vi "Convert Device Status.vi"(11 "device status":T4) -> (3 "CAN Status":T1)   [LabVIEW 2021, in "CAN RW CANsub.lvclass"]
doc: "It converts the device status to the CIF type CAN Status."
uses:
  CAN RW CANsub.lvclass
  <vilib>/CIF Foundation/CIF CAN RW Core/typedef/Communication State.ctl
  <vilib>/CIF Foundation/CIF CAN RW Core/CAN_RW_CORE.lvclass
  <vilib>/CIF Foundation/CIF CAN RW Core/typedef/Last Error.ctl
  <vilib>/CIF Foundation/CIF CAN RW Core/typedef/CAN Status.ctl
  CANsub/common/Typedefs/CANsub_Device_Status.ctl
  CANsub/common/CANsub_Common.lvlib
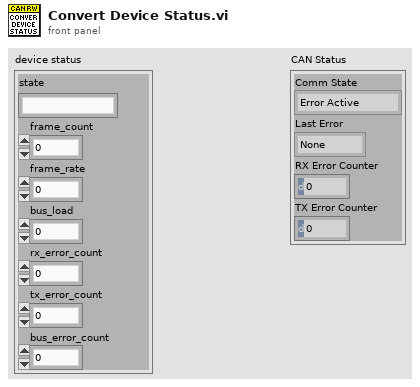
[diagram p1: front panel]
types:
  T1 = typedef "CAN_RW_CORE.lvclass/CAN Status.ctl" = cluster{"Comm State":T2, "Last Error":T3, "RX Error Counter":u8, "TX Error Counter":u8}
  T2 = typedef "CAN_RW_CORE.lvclass/Communication State.ctl" = enum16{"Error Active", "Error Passive", "Bus Off"}
  T3 = typedef "CAN_RW_CORE.lvclass/Last Error.ctl" = enum16{"None", "Stuff", "Form", "Ack", "Bit1", "Bit0", "CRC", "Unknown"}
  T4 = typedef "CANsub_Common.lvlib/CANsub_Device_Status.ctl" = cluster{"state":string, "frame_count":u32, "frame_rate":dbl, "bus_load":dbl, "rx_error_count":u32, "tx_error_count":u32, "bus_error_count":u32}
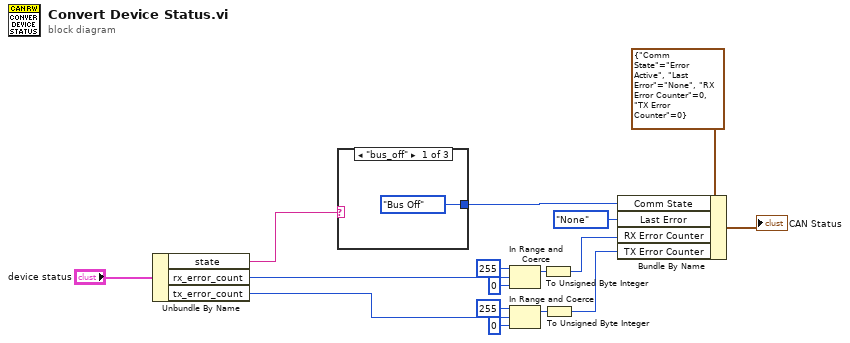
[diagram p0: block diagram]
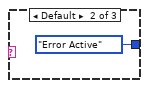
[diagram p2: hidden frame]
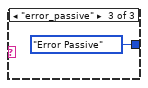
[diagram p3: hidden frame]
diagram:
  n1 = Unbundle By Name("device status") -> ("state"=w15:string, "rx_error_count"=w14:u32, "tx_error_count"=w9:u32)
  n2 = case shown="\"bus_off\"" w15 {
    tunnel: [Communication_State."Bus Off" ("Comm State") Communication_State."Error Active" ("Comm State") Communication_State."Error Passive" ("Comm State")] -> w7
    frame "bus_off" {
    }
    frame Default {
    }
    frame "error_passive" {
    }
  }
  n3 = In Range and Coerce(upper limit=u32 255, x=w14, lower limit=u32 0) -> (coerced(x)=w5:u32)  [unwired: 1 out]
  n4 = In Range and Coerce(upper limit=u32 255, x=w9, lower limit=u32 0) -> (coerced(x)=w4:u32)  [unwired: 1 out]
  n5 = To Unsigned Byte Integer(number=w5) -> (unsigned 8bit integer=w2:u8)
  n6 = To Unsigned Byte Integer(number=w4) -> (unsigned 8bit integer=w3:u8)
  n7 = Bundle By Name(cluster=T1 {"Comm State"=enum."Error Active", "Last Error"=enum."None", "RX Error Counter"=0, "TX Error Counter"=0} ("CAN Status"), "Comm State"=w7, "Last Error"=Last_Error."None", "RX Error Counter"=w2, "TX Error Counter"=w3) -> (→"CAN Status":T1)
